vi "Script Flat to Rich Oneof Conversion.vi"(5 "message element metadata":T1={"Field Name"="", "Embedded Message Name"="", "Protobuf Index"=1, "MessageElementType"=enum."StringValue", "Repeated"=FALSE, "Is in Oneof"=FALSE, "Oneof Container Name"=""}, 7 "library in":refnum<vi>, 8 "error in (no error)":errorcluster, 9 "unbundler":refnum<vi>, 10 "bundler":refnum<vi>, 11 "vi in":refnum<vi>) -> (0 "error out":errorcluster, 3 "vi out":refnum<vi>)   [LabVIEW 2019, in "gRPC Template Creation Utility.lvlib"]
uses:
  gRPC Template Creation Utility.lvlib
  TypeDefs/Message Element Metadata (Scripting).ctl
  TypeDefs/Message Element Type.ctl
  OneOf Constants/OneOfConstantsEnum.ctl
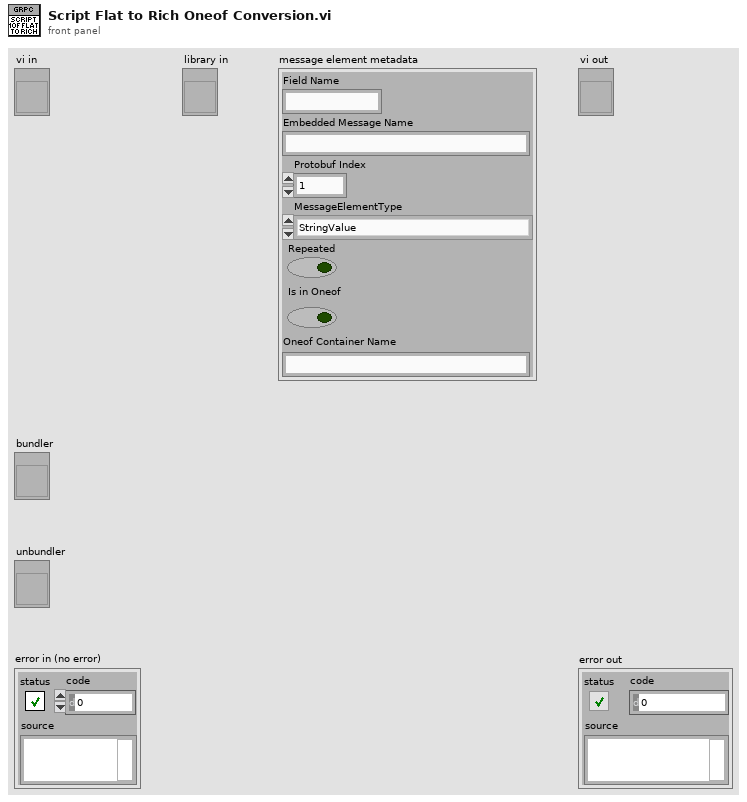
[diagram p1: front panel]
types:
  T1 = typedef "gRPC Template Creation Utility.lvlib/Message Element Metadata (Scripting).ctl" = cluster{"Field Name":string, "Embedded Message Name":string, "Protobuf Index":i32, "MessageElementType":T2, "Repeated":bool, "Is in Oneof":bool, "Oneof Container Name":string}
  T2 = typedef "gRPC Template Creation Utility.lvlib/Message Element Type.ctl" = enum32{"Int32Value", "FloatValue", "DoubleValue", "BoolValue", "StringValue", "MessageValue", "Int64Value", "UInt32Value", "UInt64Value", "EnumValue", "Bytes", "Fixed64", "Fixed32", "SFixed64", "SFixed32", "SInt64", "SInt32"}
  T3 = typedef "gRPC Template Creation Utility.lvlib/OneOfConstantsEnum.ctl" = enum16{"FlatToRichVIPrefix", "RichToFlatVIPrefix", "FlatTypeDefSuffix"}
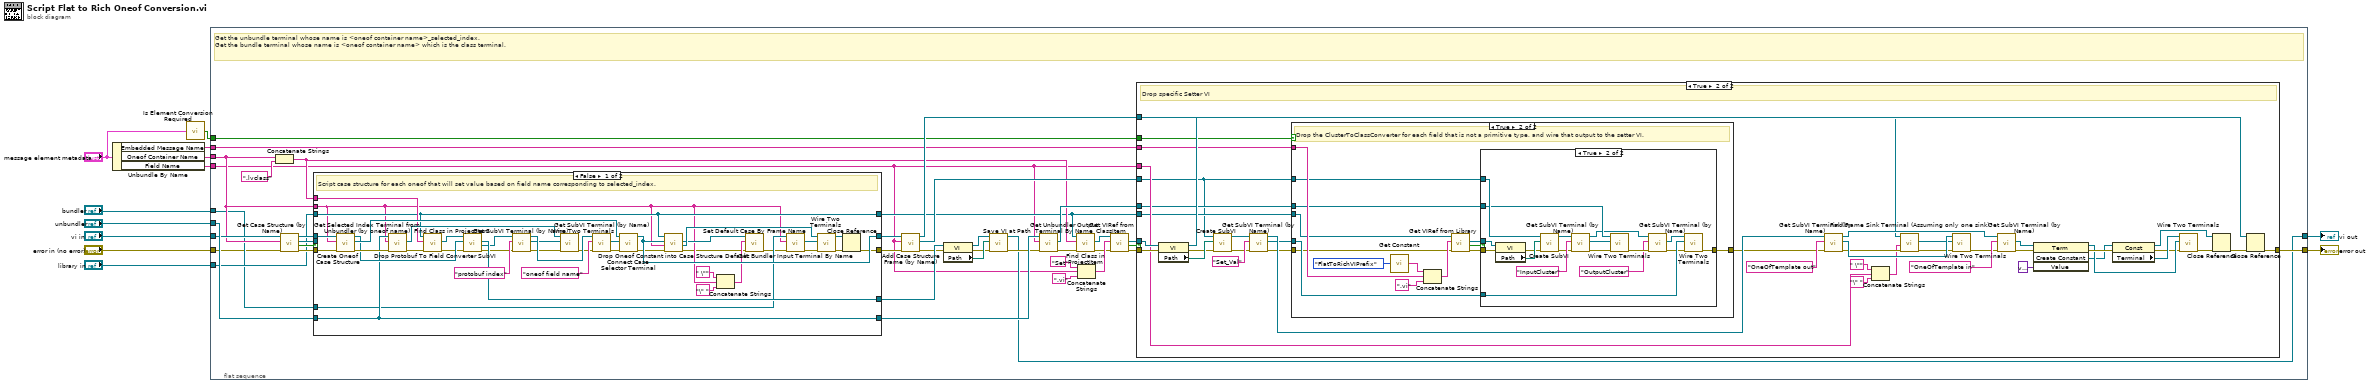
[diagram p0: block diagram]
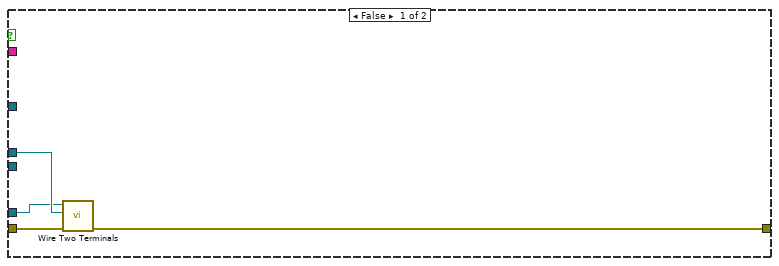
[diagram p3: hidden frame]
diagram:
  n1 = Unbundle By Name("message element metadata") -> ("Embedded Message Name"=w10:string, "Oneof Container Name"=w12:string, "Field Name"=w11:string)
  n2 = call "Is Element Conversion Required.vi"("element metadata"="message element metadata") -> ("conversion required"=w1:bool)
  n3 = flat-sequence {
    tunnel: w12 -> [w38]
    tunnel: w11 -> [w13]
    tunnel: "error in (no error)" -> [w14]
    tunnel: [w37] -> w4
    tunnel: "bundler" -> [w15]
    tunnel: "unbundler" -> [w51]
    tunnel: "vi in" -> [w50]
    tunnel: "library in" -> [w36]
    tunnel: [w30] -> w3
    tunnel: w1 -> [w24]
    tunnel: w10 -> [w23]
    frame #0 {
      # "Get the unbundle terminal whose name is <oneof container name>_selected_index.\nGet the bundle terminal whose name is <oneof container name> which is the class terminal."
      n4 = Concatenate Strings(w38, ".lvclass" ("string")) -> (w26:string)
      n5 = call "Get Case Structure (by Name).vi"("error in (no error)"=w14, "Case Structure name"=w38, "VI ref in"=w50) -> ("error out"=w44:errorcluster, "Found ?"=w48:bool, "CaseStructure out"=w45:refnum<vi>, "VI ref out"=w49:refnum<vi>)  [unwired: 5 in]
      n6 = case shown="False" w48 {
        tunnel: w51 -> [w140 w174]
        tunnel: w38 -> [w138 _]
        tunnel: w49 -> [w170 w172]
        tunnel: [w153 w175] -> w43
        tunnel: w45 -> [_ w175]
        tunnel: [w140 w174] -> w40
        tunnel: [w134 w173] -> w41
        tunnel: w44 -> [w136 w173]
        tunnel: [w166 w172] -> w34
        tunnel: w36 -> [w141 w171]
        tunnel: [w141 w171] -> w22
        tunnel: w26 -> [w142 _]
        tunnel: w15 -> [w139 _]
        frame False {
          # "Script case structure for each oneof that will set value based on field name corresponding to selected_index."
          n7 = call "Create Oneof Case Structure.vi"("error in (no error)"=w136, "Oneof Container Name"=w138, "VI in"=w170) -> ("error out"=w168:errorcluster, "CaseStructure out"=w169:refnum<vi>, "VI out"=w167:refnum<vi>)  [unwired: 6 in]
          n8 = call "Get Selected Index Terminal from Unbundler (by oneof name).vi"("error in (no error)"=w168, "Oneof Container Name"=w138, "Unbundler in"=w140) -> ("error out"=w144:errorcluster, "Terminal Refnum"=w160:refnum<vi>)  [unwired: 5 in, 2 out]
          n9 = call "Find Class in ProjectItem.vi"("error in (no error)"=w144, "Class Name"=w142, "ProjectItem in"=w141) -> ("error out"=w143:errorcluster, "LVClass out"=w145:refnum<vi>)  [unwired: 5 in, 2 out]
          n10 = call "Drop Protobuf To Field Converter SubVI.vi"("error in (no error)"=w143, "Owner VI in"=w167, "Library"=w145) -> ("error out"=w157:errorcluster, "SubVI out"=w165:refnum<vi>, "Owner VI out"=w166:refnum<vi>)  [unwired: 5 in, 1 out]
          n11 = call "Get SubVI Terminal (by Name).vi"("error in (no error)"=w157, "Terminal name"="protobuf index", "SubVI in"=w165) -> ("error out"=w156:errorcluster, "SubVI Term ref"=w159:refnum<vi>, "SubVI out"=w162:refnum<vi>)  [unwired: 5 in, 1 out]
          n12 = call "Wire Two Terminals.vi"("error in (no error)"=w156, "Sink Terminal in"=w159, "Source Terminal"=w160) -> ("error out"=w155:errorcluster)  [unwired: 7 in, 1 out]
          n13 = call "Get SubVI Terminal (by Name).vi"("error in (no error)"=w155, "Terminal name"="oneof field name", "SubVI in"=w162) -> ("error out"=w161:errorcluster, "SubVI Term ref"=w158:refnum<vi>)  [unwired: 5 in, 2 out]
          n14 = call "Connect Case Selector Terminal.vi"("error in (no error)"=w161, "Wire Source"=w158, "Case Structure in"=w169) -> ("error IO"=w152:errorcluster, "Case Structure out"=w153:refnum<vi>)  [unwired: 7 in]
          n15 = call "Drop Oneof Constant into Case Structure Default.vi"("error in (no error)"=w152, "Oneof Container Name"=w138, "CaseStructure in"=w153, "Library in"=w141) -> ("error out"=w133:errorcluster, "LVClass Constant Terminal out"=w154:refnum<vi>, "CaseStructure out"=w146:refnum<vi>)  [unwired: 4 in, 1 out]
          n16 = Concatenate Strings(" \"" ("string"), w138, "\" " ("string")) -> (w149:string)
          n17 = call "Set Default Case By Frame Name.vi"("error in (no error)"=w133, "Frame Name"=w149, "CaseStructure in"=w146) -> ("error out"=w132:errorcluster)  [unwired: 7 in, 1 out]
          n18 = call "Get Bundler Input Terminal By Name.vi"("error in (no error)"=w132, "Terminal name"=w138, "Bundler in"=w139) -> ("error out"=w135:errorcluster, "Terminal Refnum"=w137:refnum<vi>)  [unwired: 5 in, 2 out]
          n19 = call "Wire Two Terminals.vi"("error in (no error)"=w135, "Sink Terminal in"=w137, "Source Terminal"=w154) -> ("error out"=w151:errorcluster, "Source Terminal out"=w150:refnum<vi>)  [unwired: 7 in]
          n20 = Close Reference(reference=w150, error in (no error)=w151) -> (error out=w134:errorcluster)
        }
        frame True {
        }
      }
      n21 = call "Add Case Structure Frame (by Name).vi"("error in (no error)"=w41, "Frame name"=w13, "CaseStructure in"=w43) -> ("error out"=w29:errorcluster, "Case Frame"=w42:refnum<vi>, "CaseStructure out"=w35:refnum<vi>)  [unwired: 6 in]
      n22 = property class="VI"(reference=w34, error in=w29) -> (reference out=w32:refnum<vi>, error out=w28:errorcluster, "Path"=w31:path)
      n23 = call "Save VI at Path.vi"("error in (no error)"=w28, "Path"=w31, "VI in"=w32) -> ("error out"=w33:errorcluster, "VI out"=w30:refnum<vi>)  [unwired: 6 in, 1 out]
      n24 = call "Get Unbundler Output Terminal By Name.vi"("error in (no error)"=w33, "Terminal name"=w13, "Unbundler in"=w40) -> ("error out"=w25:errorcluster, "Terminal Refnum"=w39:refnum<vi>)  [unwired: 5 in, 2 out]
      n25 = call "Find Class in ProjectItem.vi"("error in (no error)"=w25, "Class Name"=w26, "ProjectItem in"=w22) -> ("error out"=w19:errorcluster, "LVClass out"=w21:refnum<vi>)  [unwired: 5 in, 2 out]
      n26 = Concatenate Strings("Set" ("string"), w13, ".vi" ("string")) -> (w20:string)
      n27 = call "Get VIRef from ClassItem.vi"("error in (no error)"=w19, "item name"=w20, "class in"=w21) -> ("error out"=w16:errorcluster, "found"=w17:bool, "vi"=w18:refnum<vi>)  [unwired: 5 in, 1 out]
      n28 = case shown="True" w17 {
        tunnel: w18 -> [_ w94]
        tunnel: w42 -> [_ w53]
        tunnel: w39 -> [_ w56]
        tunnel: w16 -> [w52 w77]
        tunnel: [w52 w73] -> w37
        tunnel: w13 -> [_ w70]
        tunnel: w35 -> [_ w69]
        tunnel: w24 -> [_ w61]
        tunnel: w23 -> [_ w60]
        tunnel: w22 -> [_ w58]
        frame False {
        }
        frame True {
          # "Drop specific Setter VI"
          n29 = property class="VI"(reference=w94, error in=w77) -> (reference out=w74:refnum<vi>, error out=w78:errorcluster, "Path"=w93:path)
          n30 = call "Create SubVI.vi"("error in (no error)"=w78, "Path"=w93, "Diagram in"=w53) -> ("error out"=w80:errorcluster, "subVI refnum"=w92:refnum<vi>)  [unwired: 7 in]
          n31 = call "Get SubVI Terminal (by Name).vi"("error in (no error)"=w80, "Terminal name"="Set_Val", "SubVI in"=w92) -> ("error out"=w57:errorcluster, "SubVI Term ref"=w55:refnum<vi>, "SubVI out"=w90:refnum<vi>)  [unwired: 5 in, 1 out]
          n32 = case shown="True" w61 {
            tunnel: w60 -> [_ w110]
            tunnel: w58 -> [_ w109]
            tunnel: w57 -> [w98 w101]
            tunnel: w56 -> [w97 w104]
            tunnel: w55 -> [w96 w103]
            tunnel: [w95 w102] -> w54
            tunnel: w53 -> [_ w105]
            frame False {
              n33 = call "Wire Two Terminals.vi"("error in (no error)"=w98, "Sink Terminal in"=w97, "Source Terminal"=w96) -> ("error out"=w95:errorcluster)  [unwired: 7 in, 1 out]
            }
            frame True {
              # "Drop the ClusterToClassConverter for each field that is not a primitive type, and wire that output to the setter VI."
              n34 = call "Get Constant.vi"("Selection"=OneOfConstantsEnum."FlatToRichVIPrefix") -> ("String"=w99:string)
              n35 = Concatenate Strings(w99, w110, ".vi" ("string")) -> (w111:string)
              n36 = call "Get VIRef from Library.vi"("error in (no error)"=w101, "item name"=w111, "library in"=w109) -> ("error out"=w106:errorcluster, "found"=w108:bool, "vi"=w107:refnum<vi>)  [unwired: 5 in, 1 out]
              n37 = case shown="True" w108 {
                tunnel: w107 -> [_ w131]
                tunnel: w106 -> [w113 w130]
                tunnel: w105 -> [_ w128]
                tunnel: w104 -> [_ w123]
                tunnel: w103 -> [_ w117]
                tunnel: [w113 w114] -> w102
                frame False {
                }
                frame True {
                  n38 = property class="VI"(reference=w131, error in=w130) -> (error out=w125:errorcluster, "Path"=w129:path)  [unwired: 1 out]
                  n39 = call "Create SubVI.vi"("error in (no error)"=w125, "Path"=w129, "Diagram in"=w128) -> ("error out"=w124:errorcluster, "subVI refnum"=w126:refnum<vi>)  [unwired: 7 in]
                  n40 = call "Get SubVI Terminal (by Name).vi"("error in (no error)"=w124, "Terminal name"="InputCluster", "SubVI in"=w126) -> ("error out"=w121:errorcluster, "SubVI Term ref"=w122:refnum<vi>, "SubVI out"=w119:refnum<vi>)  [unwired: 5 in, 1 out]
                  n41 = call "Wire Two Terminals.vi"("error in (no error)"=w121, "Sink Terminal in"=w122, "Source Terminal"=w123) -> ("error out"=w120:errorcluster)  [unwired: 7 in, 1 out]
                  n42 = call "Get SubVI Terminal (by Name).vi"("error in (no error)"=w120, "Terminal name"="OutputCluster", "SubVI in"=w119) -> ("error out"=w115:errorcluster, "SubVI Term ref"=w116:refnum<vi>)  [unwired: 5 in, 2 out]
                  n43 = call "Wire Two Terminals.vi"("error in (no error)"=w115, "Sink Terminal in"=w117, "Source Terminal"=w116) -> ("error out"=w114:errorcluster)  [unwired: 7 in, 1 out]
                }
              }
            }
          }
          n44 = call "Get SubVI Terminal (by Name).vi"("error in (no error)"=w54, "Terminal name"="OneOfTemplate out", "SubVI in"=w90) -> ("error out"=w66:errorcluster, "SubVI Term ref"=w68:refnum<vi>, "SubVI out"=w79:refnum<vi>)  [unwired: 5 in, 1 out]
          n45 = Concatenate Strings(" \"" ("string"), w70, "\" " ("string")) -> (w64:string)
          n46 = call "Find Frame Sink Terminal (Assuming only one sink).vi"("error in (no error)"=w66, "Frame Name"=w64, "CaseStructure in"=w69) -> ("error IO"=w65:errorcluster, "Terminal ref"=w67:refnum<vi>)  [unwired: 5 in, 2 out]
          n47 = call "Wire Two Terminals.vi"("error in (no error)"=w65, "Sink Terminal in"=w67, "Source Terminal"=w68) -> ("error out"=w85:errorcluster)  [unwired: 7 in, 1 out]
          n48 = call "Get SubVI Terminal (by Name).vi"("error in (no error)"=w85, "Terminal name"="OneOfTemplate in", "SubVI in"=w79) -> ("error out"=w84:errorcluster, "SubVI Term ref"=w87:refnum<vi>)  [unwired: 5 in, 2 out]
          n49 = invoke class="Term" method="Create Constant"(reference=w87, error in=w84, "Value"=variant) -> (reference out=w81:refnum<vi>, error out=w83:errorcluster, "Create Constant"=w59:refnum<vi>)  [unwired: 1 in, 1 out]
          n50 = property class="Const"(reference=w59, error in=w83) -> (reference out=w76:refnum<vi>, error out=w72:errorcluster, "Terminal"=w82:refnum<vi>)
          n51 = call "Wire Two Terminals.vi"("error in (no error)"=w72, "Sink Terminal in"=w81, "Source Terminal"=w82) -> ("error out"=w71:errorcluster)  [unwired: 7 in, 1 out]
          n52 = Close Reference(reference=w76, error in (no error)=w71) -> (error out=w75:errorcluster)
          n53 = Close Reference(reference=w74, error in (no error)=w75) -> (error out=w73:errorcluster)
        }
      }
    }
  }
  "error out" <- w4
  "vi out" <- w3
